vi "Load Config from String.vi"(6 "Fallback Name":string, 8 "error in (no error)":refnum<class "MultiErrors.lvclass">, 10 "JSON":string) -> (0 "error out":refnum<class "MultiErrors.lvclass">, 3 "Sequence Config":refnum<class "Sequence Config.lvclass">)   [LabVIEW 2023, in "VolatusSeqConfig.lvlib" / "Sequence Config.lvclass"]
uses:
  Sequence Config.lvclass
  VolatusErrorUtilities/MultiErrors/MultiErrors.lvclass
  VolatusErrorUtilities/MultiErrors/MultiErrors.lvclass/MultiErrors.ctl
  lv-cdm/CDM-Config/Config-JSON/Config-JSON.lvclass
  lv-cdm/CDM-Config/Config Manager/Config Manager.lvclass
  lv-cdm/CDM-Config/Config Element/Config Element.lvclass
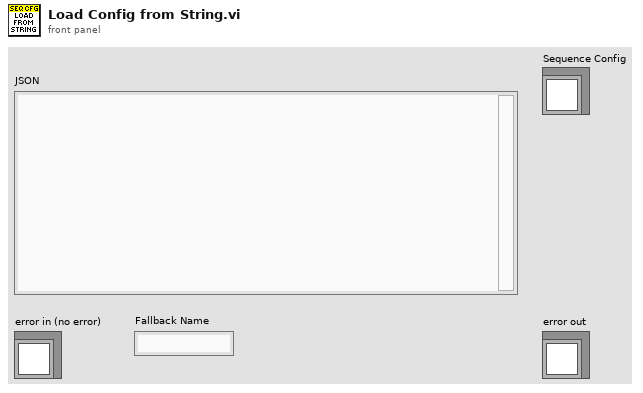
[diagram p1: front panel]
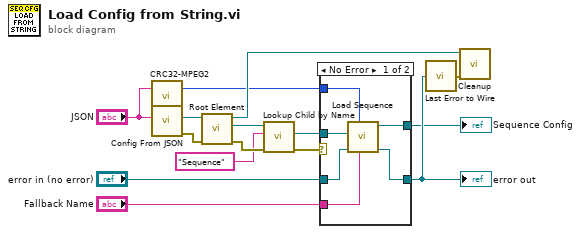
[diagram p0: block diagram]
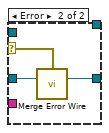
[diagram p2: hidden frame]
diagram:
  n1 = call "CRC32-MPEG2.vi"("Data In"="JSON") -> ("CRC"=w3:u32)  [unwired: 6 in]
  n2 = call "Config From JSON.vi"("JSON"="JSON") -> ("error out"=w9:errorcluster, "Config"=w12:refnum<class "Config Manager.lvclass">)  [unwired: 9 in]
  n3 = call "Root Element.vi"("error in (no error)"=w9, "Config Manager in"=w12) -> ("error out"=w13:errorcluster, "Root Element"=w11:refnum<class "Config Element.lvclass">, "Config Manager out"=w5:refnum<class "Config Manager.lvclass">)  [unwired: 7 in]
  n4 = call "Lookup Child by Name.vi"("error in (no error)"=w13, "Name"="Sequence", "Config Element in"=w11) -> ("error out"=w7:errorcluster, "Child"=w8:refnum<class "Config Element.lvclass">)  [unwired: 5 in, 2 out]
  n5 = case shown="No Error" w7 {
    selector: w7 -> [_ w23]
    tunnel: w8 -> [w21 _]
    tunnel: [w20 _] -> w6
    tunnel: w3 -> [w19 _]
    tunnel: "error in (no error)" -> [w18 w24]
    tunnel: [w17 w22] -> w15
    tunnel: "Fallback Name" -> [w16 _]
    frame No Error {
      n6 = call "Load Sequence.vi"("Fallback Name"=w16, "CRC"=w19, "error in (no error)"=w18, "Config Element"=w21) -> ("error out"=w17:refnum<class "MultiErrors.lvclass">, "Sequence Config out"=w20:refnum<class "Sequence Config.lvclass">)  [unwired: 6 in]
    }
    frame Error {
      n7 = call "Merge Error Wire.vi"("error in (no error)"=w23, "MultiErrors in"=w24) -> ("MultiErrors out"=w22:refnum<class "MultiErrors.lvclass">)  [unwired: 13 in]
    }
  }
  "error out" <- w15
  "Sequence Config" <- w6
  n8 = call "Last Error to Wire.vi"("MultiErrors in"=w15) -> ("error out"=w14:errorcluster)  [unwired: 8 in]
  n9 = call "Cleanup.vi"("error in (no error)"=w14, "Config Manager in"=w5) -> ()  [unwired: 9 in, 1 out]
